vi "Default.vi"(8 "error in (no error)":errorcluster, 11 "Channel in":refnum<class "Channel Config.lvclass">) -> (0 "error out":errorcluster, 2 "Default":string, 3 "Channel out":refnum<class "Channel Config.lvclass">)   [LabVIEW 2020, in "VolatusConfig.lvlib" / "Channel Config.lvclass"]
uses:
  Channel Config.lvclass
  C:/dev/lv20CE/relink/lv-volatus/VolatusConfig/VolatusConfigElement/VolatusConfigElement.lvclass
  VolatusConfigElement/VolatusConfigElement.lvclass/VolatusConfigElement.ctl
  Channel Config.lvclass/Channel Config.ctl
  lv-cdm/CDM-Config/Config Element/Config Element.lvclass
  VolatusConfigElement/VolatusConfigElement.lvclass
  C:/dev/lv20CE/relink/lv-volatus/VolatusConfig/Channel/Channel Config.lvclass
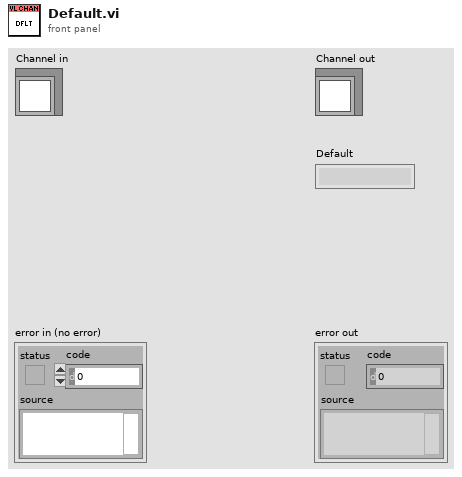
[diagram p1: front panel]
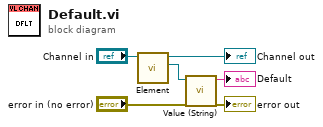
[diagram p0: block diagram]
diagram:
  n1 = call "Element.vi"("VolatusConfigElement in"="Channel in") -> ("Element"=w1:refnum<class "Config Element.lvclass">, "VolatusConfigElement out"=→"Channel out":refnum<class "Channel Config.lvclass">)  [unwired: 9 in]
  n2 = call "Value (String).vi"("Config Element in"=w1) -> ("String Value"=→"Default":string)  [unwired: 9 in, 1 out]
  "error out" <- "error in (no error)"
